vi "PR_CTICA3_PARTE_A.vi"() -> ()   [LabVIEW 2026]
panel:
  in  "Nuevo Valor":dbl
  in  "Índice":u16
  out "Indicadores":dbl[](array[numeric])
  in  "Array":dbl[](array[numeric])
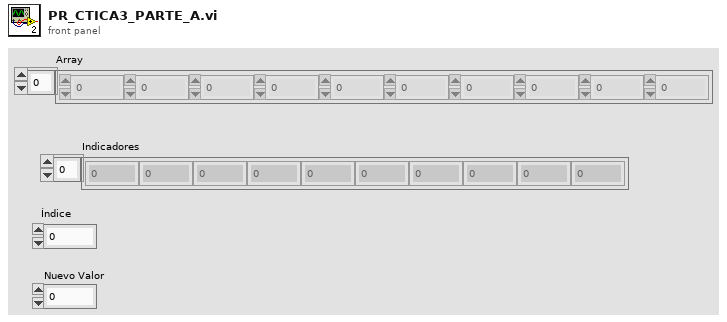
[diagram p1: front panel]
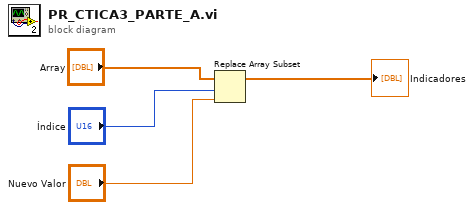
[diagram p0: block diagram]
diagram:
  n1 = Replace Array Subset(array="Array", new element="Nuevo Valor", index="Índice") -> (→"Indicadores":dbl[])
